vi "DSS-Tests-summary_common_format.vi"(11 "Common Format":T1) -> (3 "summary":dbl[](array[numeric]))   [LabVIEW 2020, in "DSS-Tests.lvlib"]
doc: "Summarises a Common Format cluster as one 1D DBL array: for each of its nine arrays in cluster order, the length, the first and the last element."
uses:
  DSS-Tests.lvlib
  Reflector/RFH-common_data_format.ctl
  Reflector/RFH-Reflection_File_Handler.lvlib
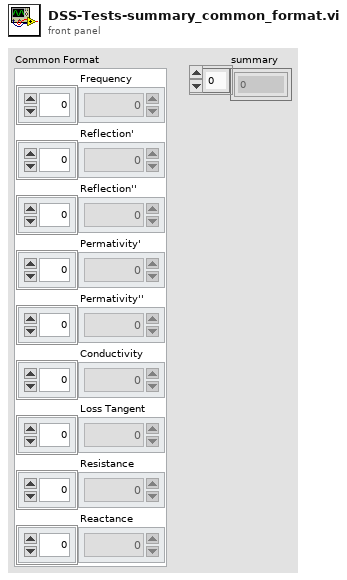
[diagram p1: front panel]
types:
  T1 = typedef "RFH-Reflection_File_Handler.lvlib/RFH-common_data_format.ctl" = cluster{"Frequency":dbl[], "Reflection'":dbl[], "Reflection''":dbl[], "Permativity'":dbl[], "Permativity''":dbl[], "Conductivity":dbl[], "Loss Tangent":dbl[], "Resistance":dbl[], "Reactance":dbl[]}
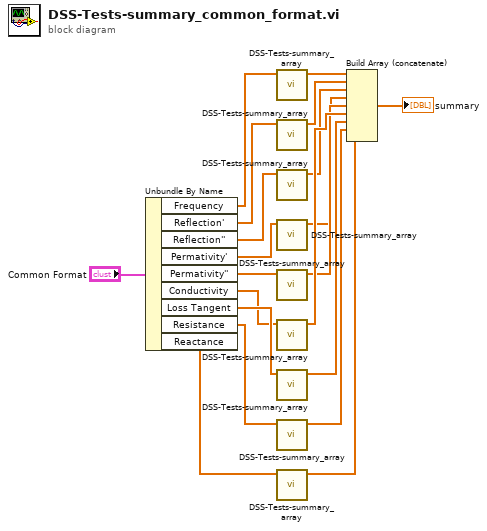
[diagram p0: block diagram]
diagram:
  n1 = Unbundle By Name("Common Format") -> ("Frequency"=w2:dbl[], "Reflection'"=w3:dbl[], "Reflection''"=w4:dbl[], "Permativity'"=w5:dbl[], "Permativity''"=w6:dbl[], "Conductivity"=w7:dbl[], "Loss Tangent"=w8:dbl[], "Resistance"=w9:dbl[], "Reactance"=w10:dbl[])
  n2 = call "DSS-Tests-summary_array.vi"("values"=w2) -> ("summary"=w11:dbl[])  [unwired: 10 in]
  n3 = call "DSS-Tests-summary_array.vi"("values"=w3) -> ("summary"=w12:dbl[])  [unwired: 10 in]
  n4 = call "DSS-Tests-summary_array.vi"("values"=w4) -> ("summary"=w13:dbl[])  [unwired: 10 in]
  n5 = call "DSS-Tests-summary_array.vi"("values"=w5) -> ("summary"=w14:dbl[])  [unwired: 10 in]
  n6 = call "DSS-Tests-summary_array.vi"("values"=w6) -> ("summary"=w15:dbl[])  [unwired: 10 in]
  n7 = call "DSS-Tests-summary_array.vi"("values"=w7) -> ("summary"=w16:dbl[])  [unwired: 10 in]
  n8 = call "DSS-Tests-summary_array.vi"("values"=w8) -> ("summary"=w17:dbl[])  [unwired: 10 in]
  n9 = call "DSS-Tests-summary_array.vi"("values"=w9) -> ("summary"=w18:dbl[])  [unwired: 10 in]
  n10 = call "DSS-Tests-summary_array.vi"("values"=w10) -> ("summary"=w19:dbl[])  [unwired: 10 in]
  n11 = Build Array (concatenate)(w11, w12, w13, w14, w15, w16, w17, w18, w19) -> (→"summary":dbl[])
